vi "RDC-Lin-Find_Capacitance.vi"(7 "Tau":dbl format="%#_6e", 10 "Open Probe reading":T1={"Frequency"=array[2001 elements], "Reflection'"=array[2001 elements], "Reflection''"=array[2001 elements], "Permativity'"=array[2001 elements], "Permativity''"=array[2001 elements], "Conductivity"=array[2001 elements], "Loss Tangent"=array[2001 elements], "Resistance"=[], "Reactance"=[]}) -> (2 "C0":dbl)   [LabVIEW 2020, in "RDC-Reflection_Data_Computation.lvlib"]
doc: "Finds the probe capacitance C0 from an open-probe Common Format cluster: corrects its reflection with Tau, computes the impedance and the capacitance."
uses:
  RDC-Reflection_Data_Computation.lvlib
  Reflector/RFH-common_data_format.ctl
  Reflector/RFH-Reflection_File_Handler.lvlib
panel:
  out "Capacitance":dbl[][](graph)
  out "Reflection":dbl[][](graph)
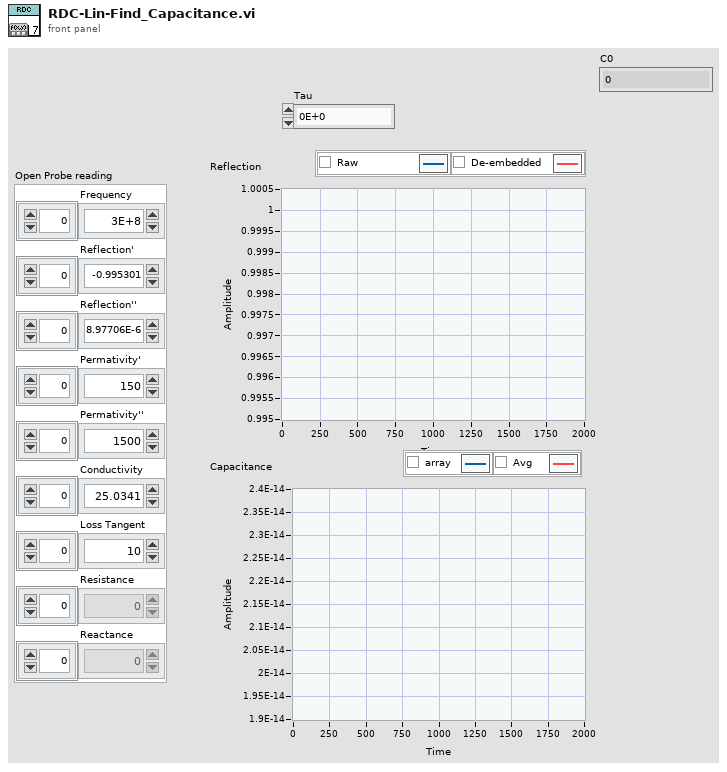
[diagram p1: front panel]
types:
  T1 = typedef "RFH-Reflection_File_Handler.lvlib/RFH-common_data_format.ctl" = cluster{"Frequency":dbl[], "Reflection'":dbl[], "Reflection''":dbl[], "Permativity'":dbl[], "Permativity''":dbl[], "Conductivity":dbl[], "Loss Tangent":dbl[], "Resistance":dbl[], "Reactance":dbl[]}
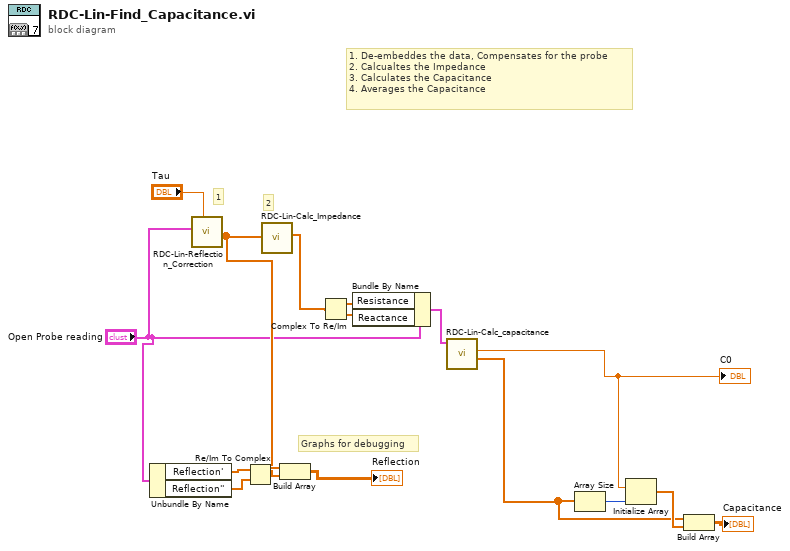
[diagram p0: block diagram]
diagram:
  # "Graphs for debugging"
  # "1. De-embeddes the data, Compensates for the probe\n2. Calcualtes the Impedance\n3. Calculates the Capacitance\n4. Averages the Capacitance"
  # "2"
  # "1"
  n1 = Unbundle By Name("Open Probe reading") -> ("Reflection'"=w14:dbl[], "Reflection''"=w13:dbl[])
  n2 = call "RDC-Lin-Reflection_Correction.vi"("Tau"="Tau", "Measured"="Open Probe reading") -> ("Reflection Tip"=w11:cdb[])  [unwired: 8 in, 1 out]
  n3 = Re/Im To Complex(1:w13, 2:w14) -> (0:w12:cdb[])
  n4 = call "RDC-Lin-Calc_Impedance.vi"("Reflection Tip"=w11) -> ("Impedance"=w4:cdb[])  [unwired: 9 in, 1 out]
  n5 = Build Array(w12, w11) -> (→"Reflection":cdb[][])
  n6 = Complex To Re/Im(x + iy=w4) -> (x=w6:dbl[], y=w5:dbl[])
  n7 = Bundle By Name(cluster="Open Probe reading", "Resistance"=w6, "Reactance"=w5) -> (w3:T1)
  n8 = call "RDC-Lin-Calc_capacitance.vi"("Open Probe reading"=w3) -> ("Cap array"=w2:dbl[], "C0"=w1:dbl)  [unwired: 9 in]
  "C0" <- w1
  n9 = Array Size(array=w2) -> (size(s)=w15:i32)
  n10 = Initialize Array(w1, w15) -> (w9:dbl[])
  n11 = Build Array(w2, w9) -> (→"Capacitance":dbl[][])
